vi "BNAL assembly.vi"(7 "Right Read MIN":i32=5, 8 "Mx Right No":i32[](array[numeric]), 9 "Seq ENo":i32[](array[numeric]), 10 "Seq SNo":i32[](array[numeric]), 11 "Cutted Sample Sequence":string) -> (0 "Long Signal#":i32, 3 "Long Assembly":bool[][](array[boolean]))   [LabVIEW 2018]
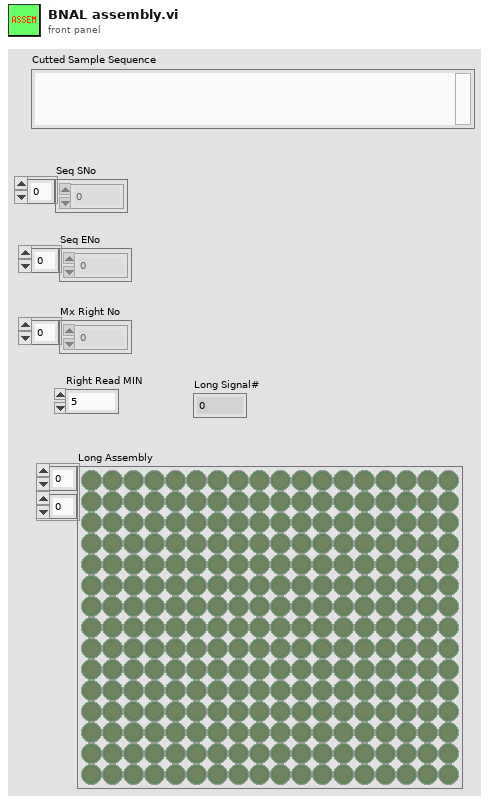
[diagram p1: front panel]
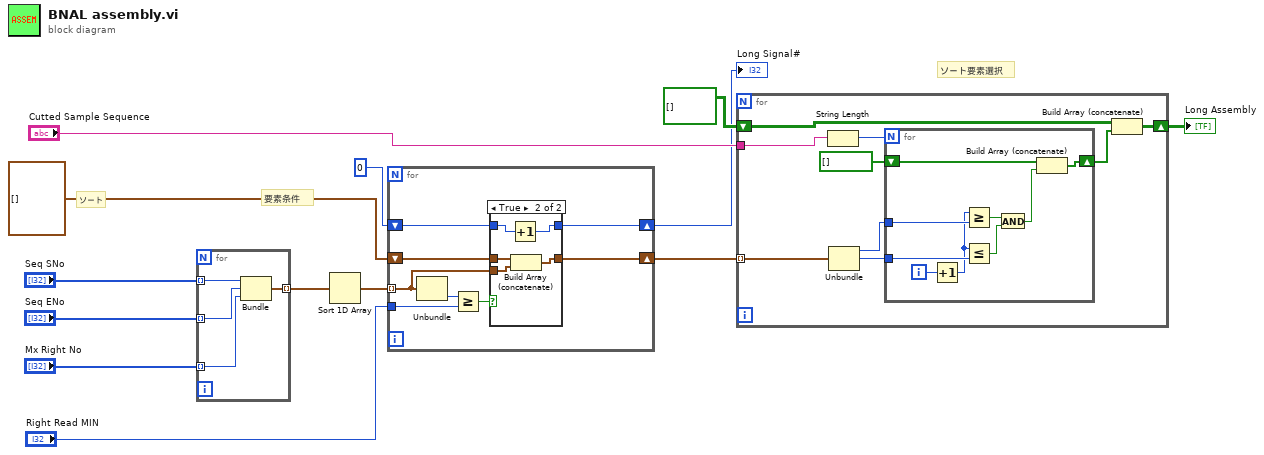
[diagram p0: block diagram]
diagram:
  # "要素条件"
  # "ソート"
  # "ソート要素選択"
  n1 = for {
    tunnel: [w17] -> w13 mode=indexing
    tunnel: "Seq SNo" -> [w16] mode=indexing
    tunnel: "Seq ENo" -> [w15] mode=indexing
    tunnel: "Mx Right No" -> [w14] mode=indexing
    n2 = Bundle(w16, w15, w14) -> (w17:cluster{i32, i32, i32})  [unwired: 1 in]
  }
  n3 = Sort 1D Array(array=w13) -> (sorted array=w11:cluster{i32, i32, i32}[])
  n4 = for {
    tunnel: w11 -> [w25] mode=indexing
    shift-right: [w24] -> w5
    shift-left: cluster{i32, "offset past number":i32, i32}[] [] -> [w23]
    tunnel: "Right Read MIN" -> [w21]
    shift-right: [w19] -> w6
    shift-left: 0 -> [w20]
    n5 = Unbundle(w25) -> (w18:i32)  [unwired: 2 out]
    n6 = Greater Or Equal?(x=w18, y=w21) -> (x >= y?=w22:bool)
    n7 = case shown="True" w22 {
      tunnel: w25 -> [_ w28]
      tunnel: [w27 w32] -> w24
      tunnel: w23 -> [w27 w31]
      tunnel: w20 -> [w26 w30]
      tunnel: [w26 w29] -> w19
      frame False {
      }
      frame True {
        n8 = Increment(x=w30) -> (x+1=w29:i32)
        n9 = Build Array (concatenate)(w31, w28) -> (w32:cluster{i32, "offset past number":i32, i32}[])
      }
    }
  }
  "Long Signal#" <- w6
  n10 = for {
    tunnel: w5 -> [w41] mode=indexing
    tunnel: "Cutted Sample Sequence" -> [w40]
    shift-right: [w36] -> w9
    shift-left: bool[][] [] -> [w35]
    n11 = String Length(string=w40) -> (length=w39:i32)
    n12 = Unbundle(w41) -> (w34:i32, "offset past number"=w33:i32)  [unwired: 1 out]
    n13 = for {
      N: w39 -> [_]
      tunnel: w34 -> [w43]
      tunnel: w33 -> [w45]
      shift-right: [w50] -> w37
      shift-left: bool[] [] -> [w49]
      i -> [w44]
      n14 = Increment(x=w44) -> (x+1=w42:i32)
      n15 = Greater Or Equal?(x=w42, y=w43) -> (x >= y?=w48:bool)
      n16 = Less Or Equal?(x=w42, y=w45) -> (x <= y?=w46:bool)
      n17 = And(x=w48, y=w46) -> (x .and. y?=w47:bool)
      n18 = Build Array (concatenate)(w49, w47) -> (w50:bool[])
    }
    n19 = Build Array (concatenate)(w35, w37) -> (w36:bool[][])
  }
  "Long Assembly" <- w9
